vi "4.3 Arguments - Safe Arguments if it contains key words of CSM.vi"() -> ()   [LabVIEW 2017]
doc: "#### Overview\n\nDemonstrates how to pass strings containing special characters as arguments.\n\n#### Introduction\n\nSince CSM uses text descriptions as arguments, parsing errors occur if the argument contains reserved CSM keywords. To solve this, CSM provides APIs to convert special characters in unsafe strings into safe strings for use in arguments.\n\n<b>Application Scenario</b>: Passing strings containing special characters.\n\n#### Steps\n\n- Step1: Demonstrate converting an unsafe string to a safe string and obtaining the CSM-Argument Type.\n- Step2: Demonstrate using a Windows file path as an argument.\n- Step3: Demonstrate using a URL as an argument."
uses:
  user.lib/_NEVSTOP/Communicable State Machine(CSM)/AdvanceAPI/CSM - Keywords.vi
  user.lib/_NEVSTOP/Communicable State Machine(CSM)/Communicable State Machine.lvlib
panel:
  out "equal?":bool
  in  "Argument String 3":string="https://github.com/NEVSTOP-LAB/Communicable-State-Machine"
  out "Safe Argument String 3":string="https:%2F%2Fgithub.com/NEVSTOP-LAB/Communicable-State-Machine"
  out "Safe Argument String 2":string="c:\\abc\\def.txt"
  in  "Argument String 2":string="c:\\abc\\def.txt"
  out "Safe Argument String":string="eaasdf%2D%3Efqwvrf%2D%26#%0Adddd\\\\\\\\\\not comments%0A%2F%2Fadcd\\\\de/assfd%0A%2C %5B%3B%5D%0A%2D%40asdfvq%3C%2D1234"
  out "Origin Argument String":string="eaasdf->fqwvrf-&#\ndddd\\\\\\\\\\not comments\n//adcd\\\\de/assfd\n, [;]\n-@asdfvq<-1234"
  in  "Argument String":string="eaasdf->fqwvrf-&#\ndddd\\\\\\\\\\not comments\n//adcd\\\\de/assfd\n, [;]\n-@asdfvq<-1234"
  # "#CSM-Example Overview\n\nDemonstrates how to pass strings containing special characters as arguments."
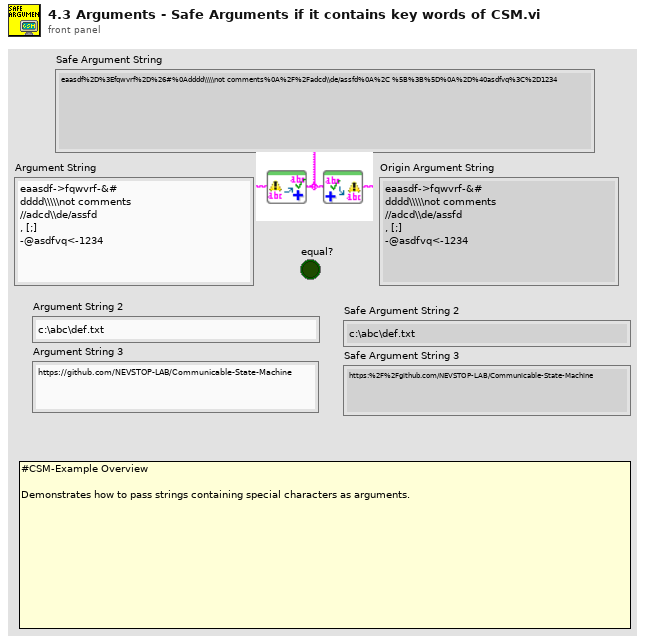
[diagram p1: front panel]
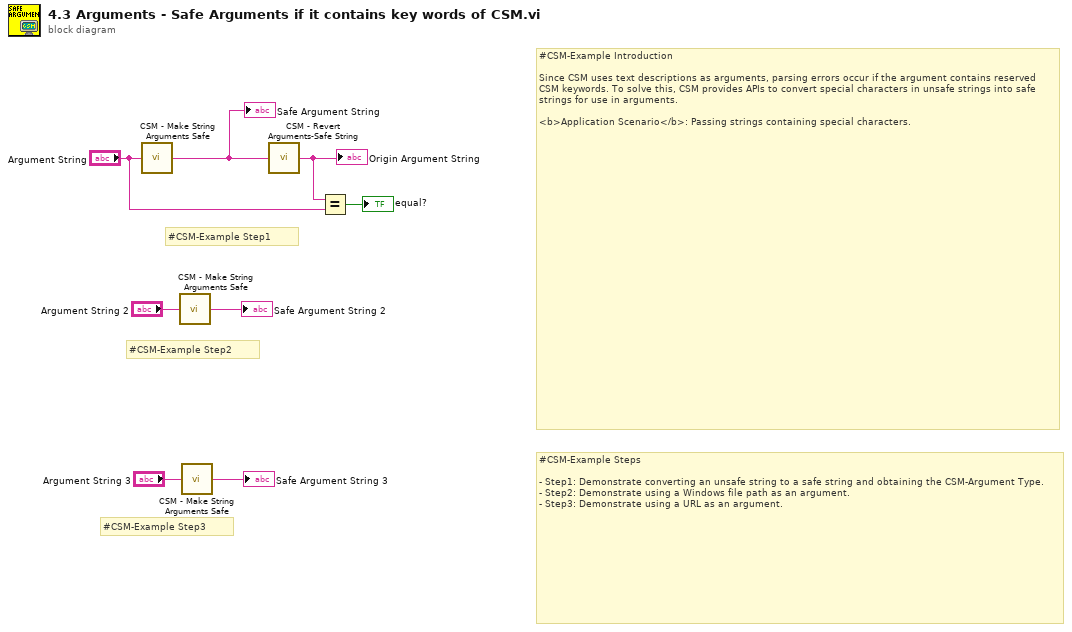
[diagram p0: block diagram]
diagram:
  # "#CSM-Example Step1"
  # "#CSM-Example Step2"
  # "#CSM-Example Step3"
  # "#CSM-Example Steps\n\n- Step1: Demonstrate converting an unsafe string to a safe string and obtaining the CSM-Argument Type.\n- Step2: Demonstrate using a Windows file path as an argument.\n- Step3: Demonstrate using a URL as an argument."
  # "#CSM-Example Introduction\n\nSince CSM uses text descriptions as arguments, parsing errors occur if the argument contains reserved CSM keywords. To solve this, CSM provides APIs to convert special characters in unsafe strings into safe strings for use in arguments.\n\n<b>Application Scenario</b>: Passing strings containing special characters."
  n1 = call "CSM - Make String Arguments Safe.vi"("Argument String"="Argument String") -> ("Safe Argument String"=w4:string)  [unwired: 8 in]
  "Safe Argument String" <- w4
  n2 = call "CSM - Make String Arguments Safe.vi"("Argument String"="Argument String 2") -> ("Safe Argument String"=→"Safe Argument String 2":string)  [unwired: 8 in]
  n3 = call "CSM - Make String Arguments Safe.vi"("Argument String"="Argument String 3") -> ("Safe Argument String"=→"Safe Argument String 3":string)  [unwired: 8 in]
  n4 = call "CSM - Revert Arguments-Safe String.vi"("Safe Argument String"=w4) -> ("Origin Argument String"=w2:string)  [unwired: 8 in]
  "Origin Argument String" <- w2
  n5 = Equal?(x=w2, y="Argument String") -> (x = y?=→"equal?":bool)
